vi "calculate_wildcards_for_shared_library_file.vi"(8 "error in":errorcluster, 11 "Shared Library Path":path) -> (0 "error out":errorcluster, 2 "sibling shared libraries":path[](array[path]), 3 "Shared Library Path with wildcards":path)   [LabVIEW 2020, in "vi_package_building_extensions.lvlib" / "fix_shared_library_wildcards.lvlib"]
uses:
  fix_shared_library_wildcards.lvlib
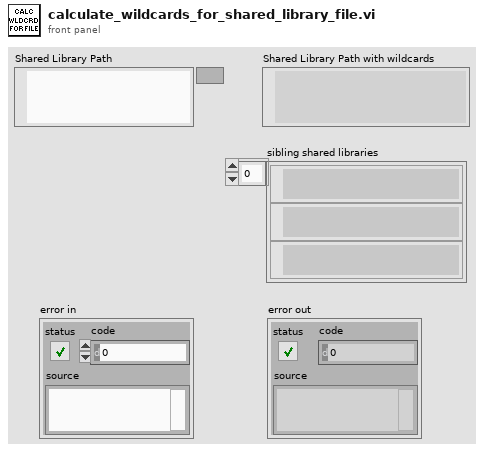
[diagram p1: front panel]
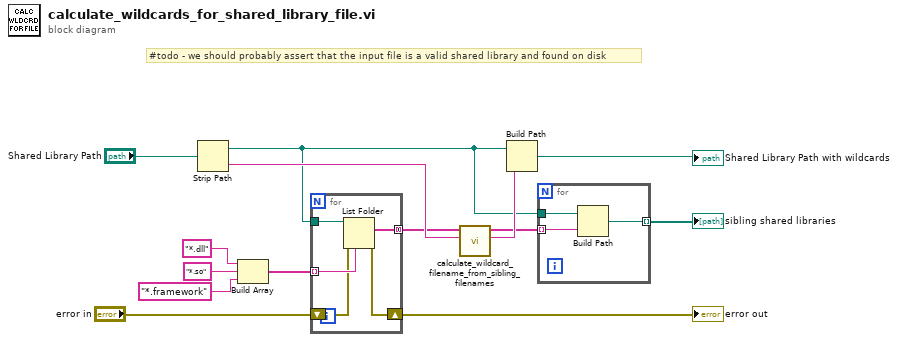
[diagram p0: block diagram]
diagram:
  # "#todo - we should probably assert that the input file is a valid shared library and found on disk"
  n1 = Strip Path(path="Shared Library Path") -> (stripped path=w4:path, name=w14:string)
  n2 = Build Array("*.dll" ("pattern"), "*.so" ("pattern"), "*.framework" ("pattern")) -> (w11:string[])
  n3 = for {
    tunnel: w11 -> [w18] mode=indexing
    tunnel: w4 -> [w19]
    tunnel: [w17] -> w13 mode=concatenating
    shift-right: [w16] -> w2
    shift-left: "error in" -> [w15]
    n4 = List Folder(path=w19, pattern=w18, error in=w15) -> (filenames=w17:string[], error out=w16:errorcluster)  [unwired: 1 in, 2 out]
  }
  "error out" <- w2
  n5 = call "calculate_wildcard_filename_from_sibling_filenames.vi"("shared library filename"=w14, "sibling filenames"=w13) -> ("wildcard filename"=w7:string, "sibling shared libraries"=w5:string[])  [unwired: 8 in]
  n6 = Build Path(base path=w4, name or relative path=w7) -> (appended path=→"Shared Library Path with wildcards":path)
  n7 = for {
    tunnel: w5 -> [w22] mode=indexing
    tunnel: w4 -> [w21]
    tunnel: [w20] -> w3 mode=indexing
    n8 = Build Path(base path=w21, name or relative path=w22) -> (appended path=w20:path)
  }
  "sibling shared libraries" <- w3
